vi "Config_Encode.vi"(8 "error in (no error)":errorcluster={"status"=FALSE, "code"=0, "source"="\"\""}, 10 "TestDefinition":string, 11 "RigDefinition":string) -> (0 "error out":errorcluster={"status"=FALSE, "code"=0, "source"="\"\""}, 2 "status ok":bool, 3 "Raw package bytes":string)   [LabVIEW 2026]
doc: "INTENT: Encode configuration tree into versioned serialized package. LOGIC: Serialize configuration into structured JSON/binary package with schema manifest"
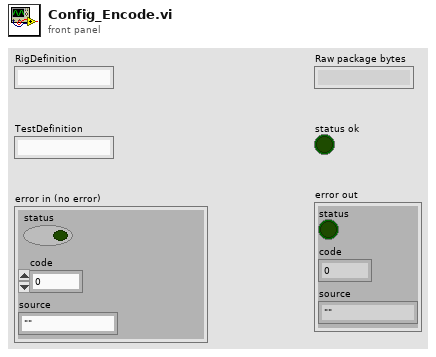
[diagram p1: front panel]
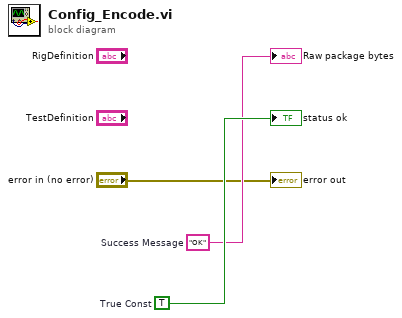
[diagram p0: block diagram]
diagram:
  w3 = TRUE  # True Const
  w2 = "OK"  # Success Message
  "Raw package bytes" <- w2
  "status ok" <- w3
  "error out" <- "error in (no error)"
